vi "YAV_Init.vi"(0 "Device Index":u32, 5 "WriteParam":u8[](array[numeric])=[7] format="%.0x", 7 "CMD":u8=170 format="%.0x", 9 "error in":errorcluster caption="错误输入（无错误）") -> (4 "Device Count":u32, 6 "Device ID":u32 format="%.0x", 8 "Hardware Valid":bool, 10 "error out":errorcluster caption="错误输出")   [LabVIEW 2020]
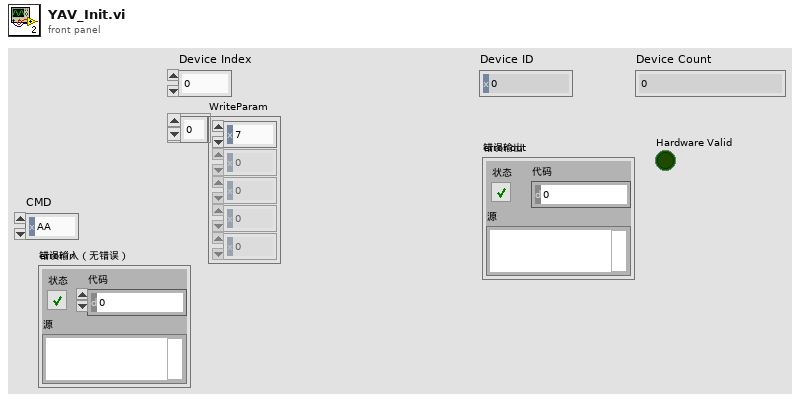
[diagram p1: front panel]
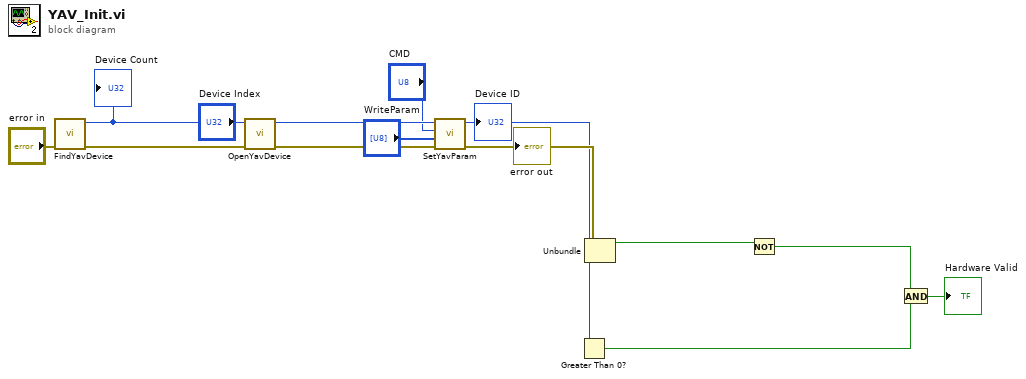
[diagram p0: block diagram]
diagram:
  n1 = call "FindYavDevice.vi"("错误输入（无错误）"="error in") -> ("错误输出"=w14:errorcluster, "设备数量"=w5:u32)  [unwired: 8 in, 1 out]
  "Device Count" <- w5
  n2 = call "OpenYavDevice.vi"("错误输入（无错误）"=w14, "ID"="Device Index") -> ("错误输出"=w13:errorcluster, "ID"=w12:u32)  [unwired: 8 in]
  n3 = call "SetYavParam.vi"("错误输入（无错误）"=w13, "WriteParam"="WriteParam", "CMD"="CMD", "ID"=w12) -> ("错误输出"=w6:errorcluster, "ID"=→"Device ID":u32)  [unwired: 6 in]
  "error out" <- w6
  n4 = Greater Than 0?(x=w5) -> (x > 0?=w3:bool)
  n5 = Unbundle(w6) -> ("status"=w4:bool)  [unwired: 2 out]
  n6 = Not(x=w4) -> (.not. x?=w2:bool)
  n7 = And(x=w2, y=w3) -> (x .and. y?=→"Hardware Valid":bool)
